vi "Curve Editor(CSM).vi"() -> ()   [LabVIEW 2020, in "Curve Editor.lvlib"]
doc: "------------- lvcsm -------------\n[CSMStates]\nItem 0 = \"Event Structure\"\nItem 1 = \"Idle\"\nItem 2 = \"CSM Documentation\"\nItem 3 = \"VI Reference\"\nItem 4 = \"Error Handler\"\nItem 5 = \"Critical Error\"\nItem 6 = \"Target Timeout Error\"\nItem 7 = \"Target Error\"\nItem 8 = \"Async Response\"\nItem 9 = \"Response\"\nItem 10 = \"Async Message Posted\"\nItem 11 = \"Initialize Core Data\"\nItem 12 = \"Exit\"\nItem 13 = \"Data: Initialize\"\nItem 14 = \"Data: Cleanup\"\nItem 15 = \"Events: Register\"\nItem 16 = \"Events: Unregister\"\nItem 17 = \"UI: Initialize\"\nItem 18 = \"UI: Cursor Set\"\nItem 19 = \"UI: Front Panel State\"\nItem 20 = \"Macro: Initialize\"\nItem 21 = \"Macro: Exit\"\nItem 22 = \"Action: Write File\"\nItem 23 = \"Action: Read File\"\nItem 24 = \"Action: Draw Plot\"\nItem 25 = \"Action: Handle Unsaved Porcess\"\nItem 26 = \"Action: Open File\"\nItem 27 = \"Action: Save File\"\nItem 28 = \"Action: New File\"\nItem 29 = \"Action: Edit Item\"\n\n[CSMStatus]\nItem 0 = \"Error Occurred@Error Handler\""
uses:
  Curve Editor.lvlib
  Curve Editor/User Data--cluster.ctl
  <vilib>/Utility/miscctls.llb/LVPointTypeDef.ctl
  7b0969bd-7955-4222-98c9-53128525ee30.vi
  183b1dfd-394f-40bc-8548-5665fe87f6d3.vi
  54737b30-700e-483c-a5e2-87d6bca6278c.vi
  <userlib>/_NEVSTOP/Communicable State Machine(CSM)/AdvanceAPI/CSM - Revert Arguments-Safe String.vi
  <userlib>/_NEVSTOP/Communicable State Machine(CSM)/_Shared/Trim Single-line Text.vi
  <userlib>/_NEVSTOP/Communicable State Machine(CSM)/AdvanceAPI/CSM - Make String Arguments Safe.vi
  <userlib>/_NEVSTOP/Communicable State Machine(CSM)/AdvanceAPI/CSM - Break Down Multiple States String.vi
  <userlib>/_NEVSTOP/Communicable State Machine(CSM)/AdvanceAPI/CSM - Compact Multiple States.vi
  <userlib>/_NEVSTOP/Communicable State Machine(CSM)/AdvanceAPI/CSM - Keywords.vi
  <userlib>/_NEVSTOP/Communicable State Machine(CSM)/addons/API-String-Arugments-Support/_Support/Data To API String Arguments.vi
  <vilib>/Utility/file.llb/Read Delimited Spreadsheet (string).vi
  <userlib>/_NEVSTOP/Communicable State Machine(CSM)/addons/API-String-Arugments-Support/_Support/Convert API String Arguments to Data(variant).vi
  <userlib>/_NEVSTOP/Communicable State Machine(CSM)/Communicable State Machine.lvlib
panel:
  out "State History":string
  in  "Tab Control":enum32{"Page 1"}(tab)
  in  "动作列表框":i32(listbox) caption="曲线片段"
  in  "循环树形":string(tree) caption="循环编辑"
  in  "打开按钮":bool
  in  "保存按钮":bool
  in  "另存为按钮":bool
  in  "新建按钮":bool
  out "曲线预览":cluster{"X":dbl[], "Y":dbl[]}(graph)
  out "总时长[秒]":dbl format="%.2f"
  in  "Name (\"\" to Use UUID)":string="Curve Editor"
  # "曲线编辑"
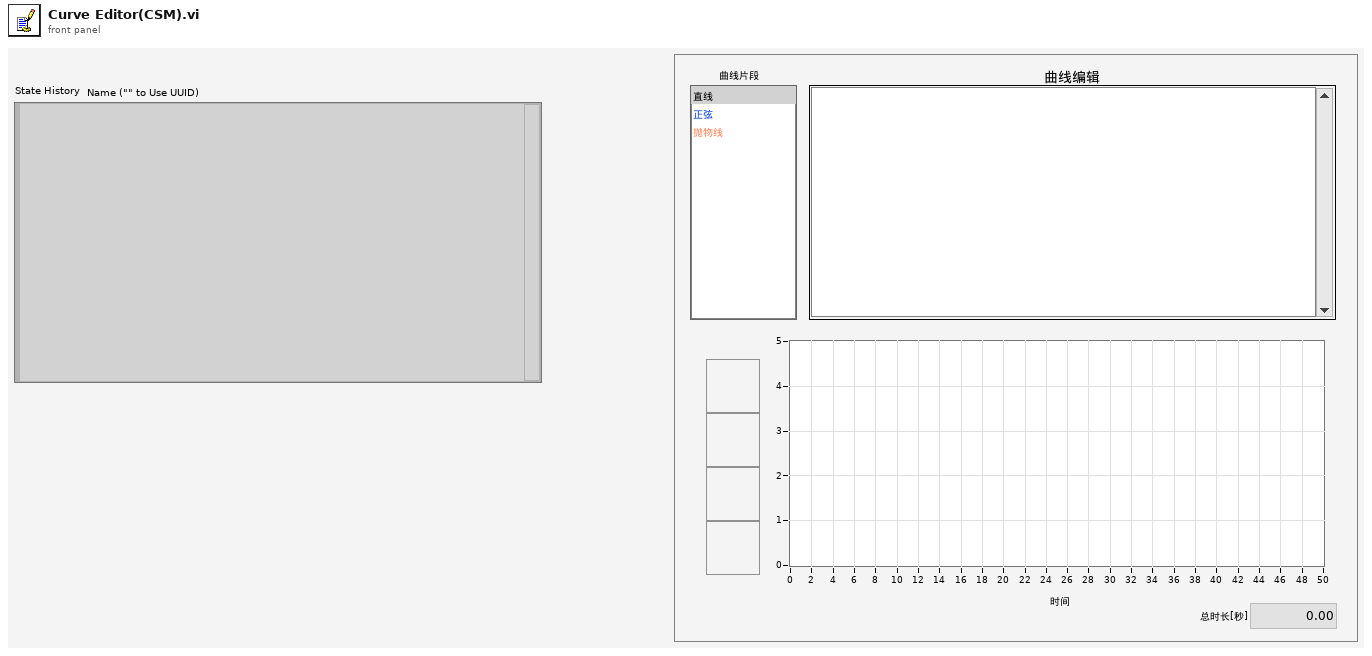
[diagram p1: front panel]
types:
  T1 = enum32{"Invalid", "Standard", "Closed", "Hidden", "Minimized", "Maximized"}
  T2 = enum32{"invalid app kind", "Development System", "Run Time System", "Student Edition", "Embedded LabVIEW", "Evaluation", "Custom"}
  T3 = cluster{"开始路径":path, "默认名称":string, "类型(后缀名)":string, "类型标签":string}
  T4 = typedef "LVPointTypeDef.ctl" = cluster{"Horizontal":i16, "Vertical":i16}
  T5 = enum16{"open", "replace", "create", "open or create", "replace or create", "replace or create with confirmation"}
  T6 = typedef "Communicable State Machine.lvlib/_CSM_Response Source Message.ctl" = cluster{"‘State":string, "’Arguments":string, "’Error":errorcluster}
  T7 = typedef "LVPoint32TypeDef.ctl" = cluster{"Horizontal":i32, "Vertical":i32}
  T8 = typedef "Curve Editor.lvlib/User Data--cluster.ctl" = cluster{"窗体标题":string, "文件参数":cluster{"默认路径":path, "默认名称":string, "类型(后缀名)":string, "类型标签":string}, "颜色符号列表":cluster{"项名":string, "颜色":u32, "符号":i32}[], "循环数组":string[], "文件路径":path, "文件已保存":bool, "存盘提醒":bool}
  T9 = cluster{"Core":cluster{"Current VI Reference":refnum<vi>, "Close Panel on Exit?":bool}, "User Data":T8}
  T10 = cluster{"Current VI Reference":refnum<vi>, "Close Panel on Exit?":bool}
  T11 = cluster{"默认路径":path, "默认名称":string, "类型(后缀名)":string, "类型标签":string}
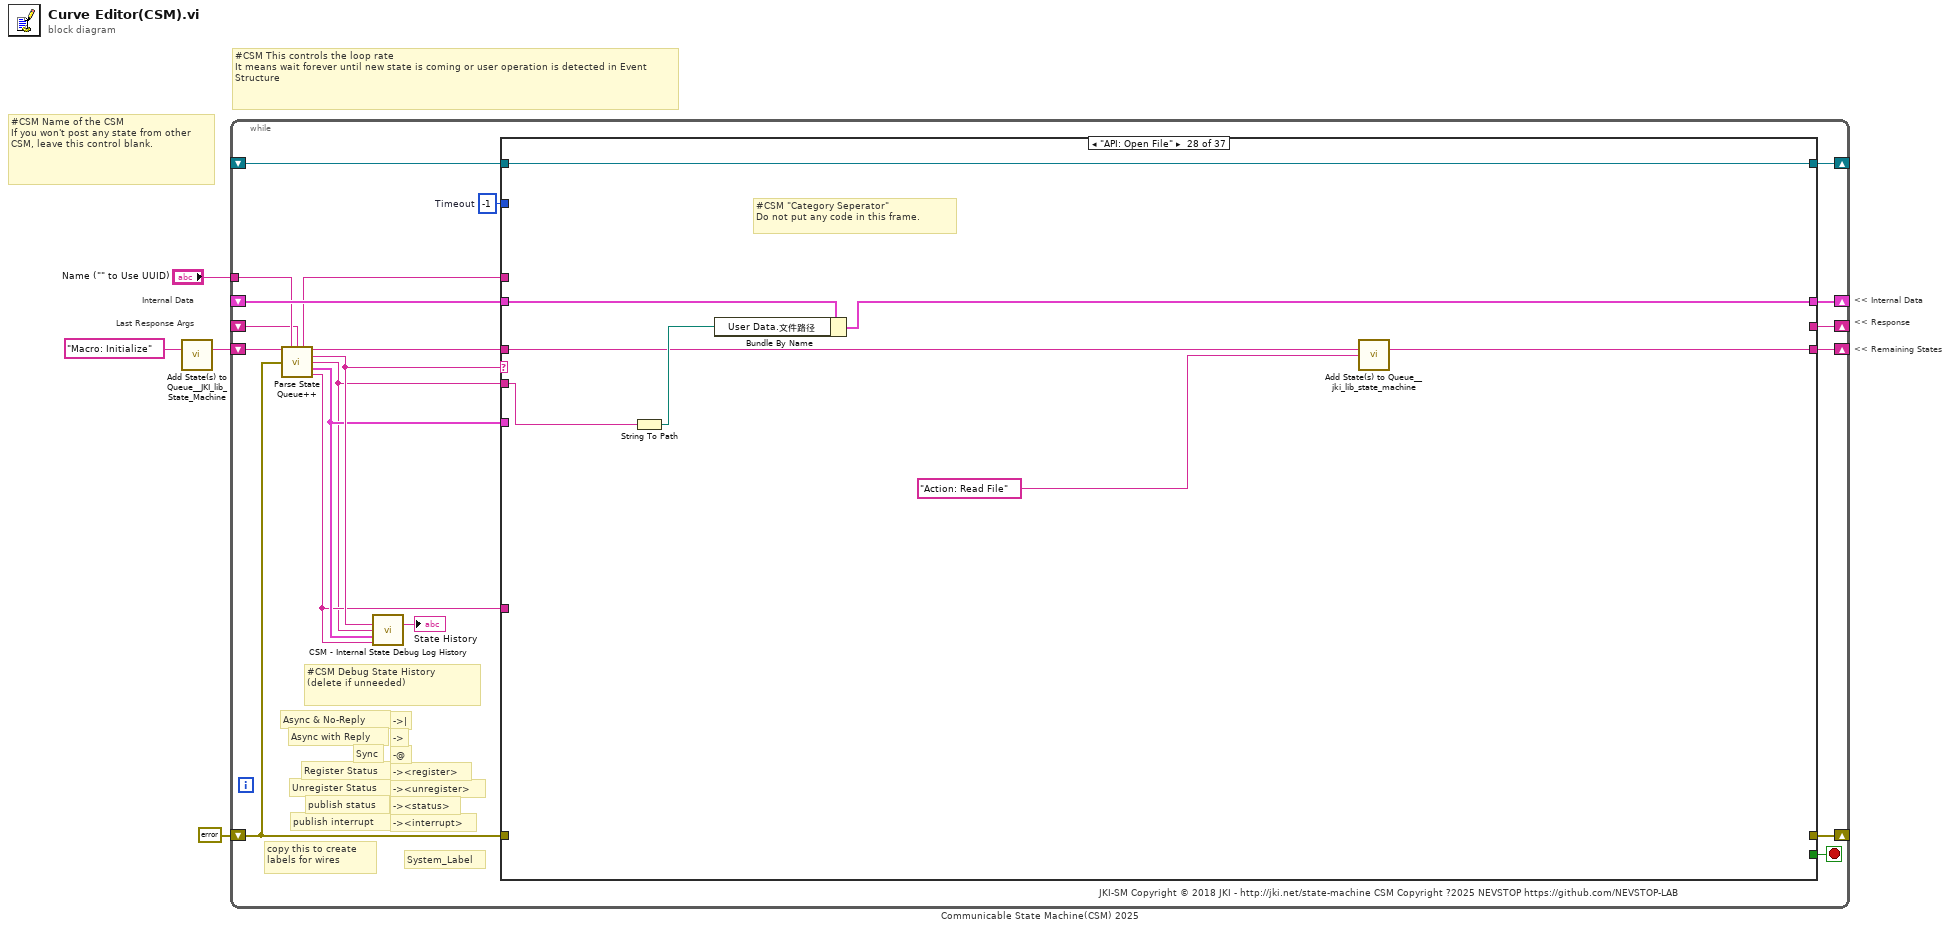
[diagram p0: block diagram]
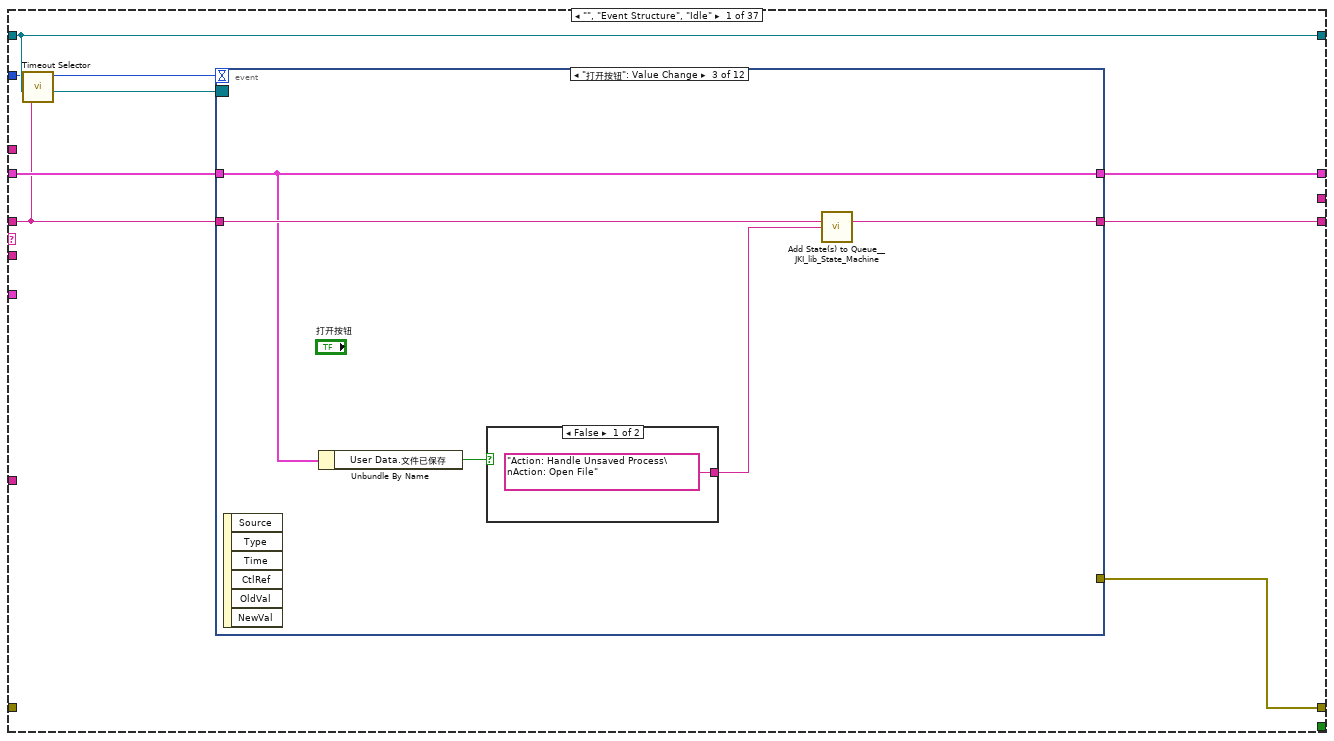
[diagram p2: hidden frame]
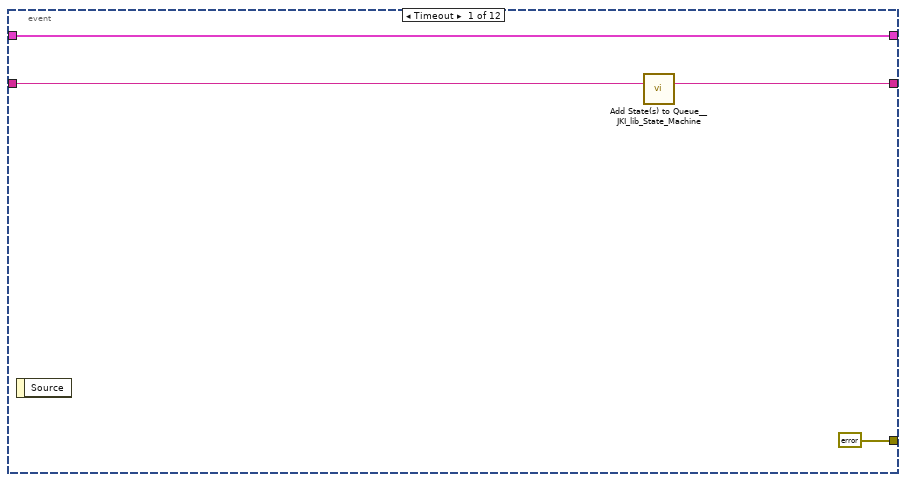
[diagram p3: hidden frame]
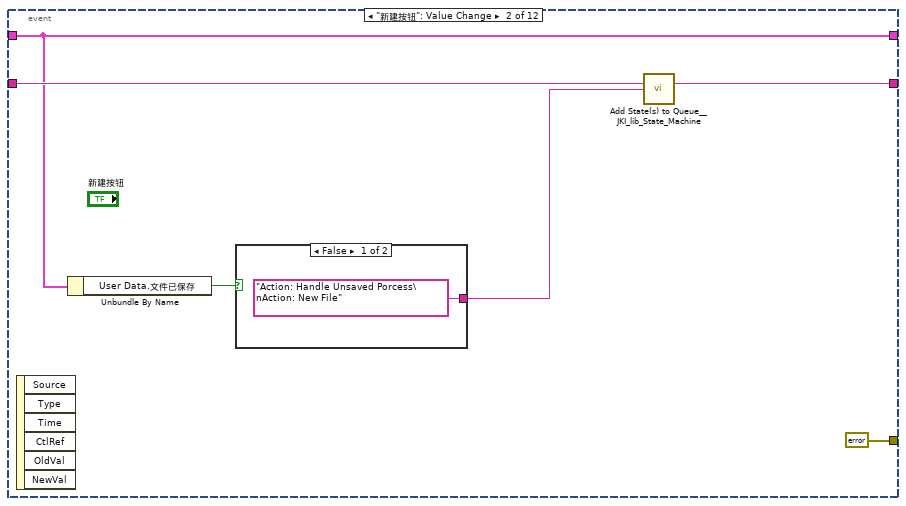
[diagram p4: hidden frame]
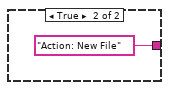
[diagram p5: hidden frame]
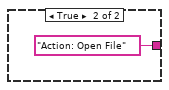
[diagram p6: hidden frame]
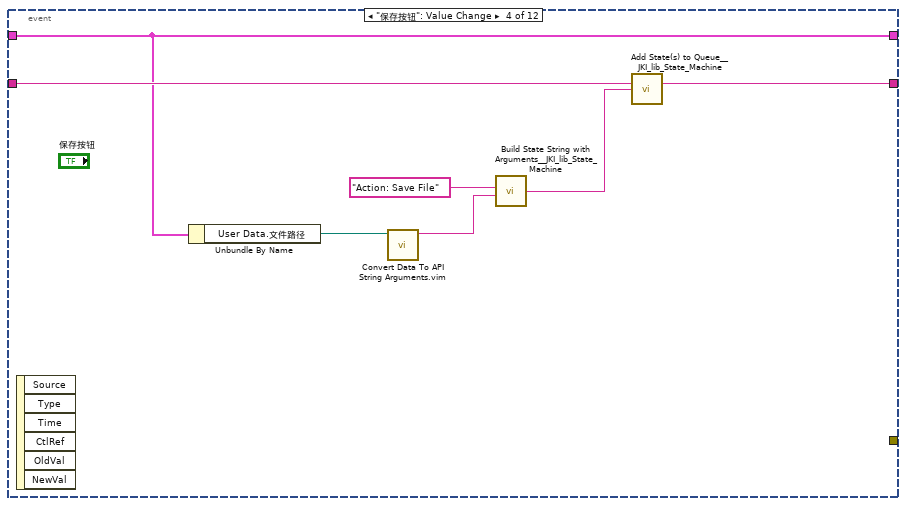
[diagram p7: hidden frame]
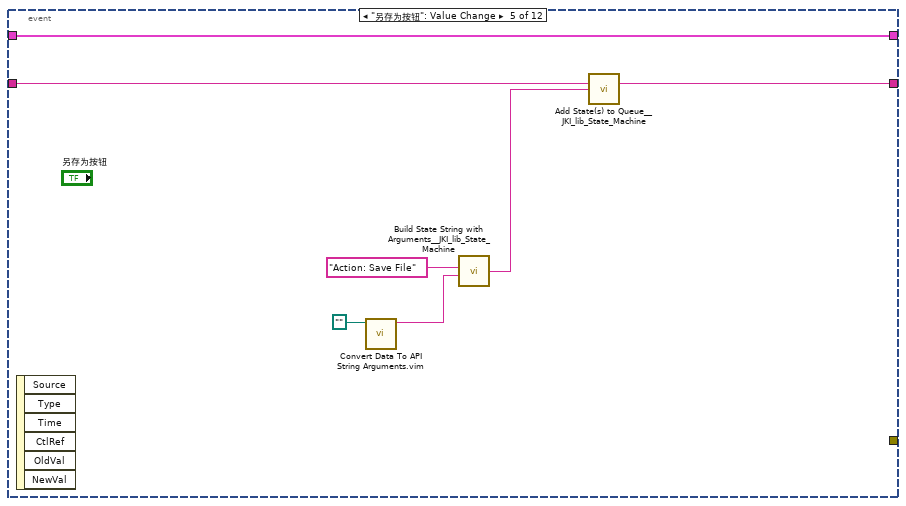
[diagram p8: hidden frame]
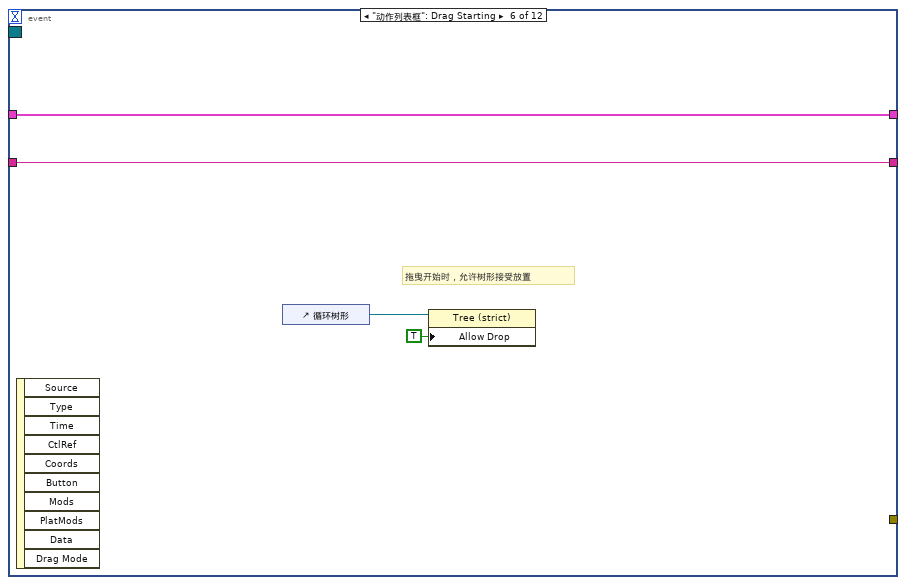
[diagram p9: hidden frame]
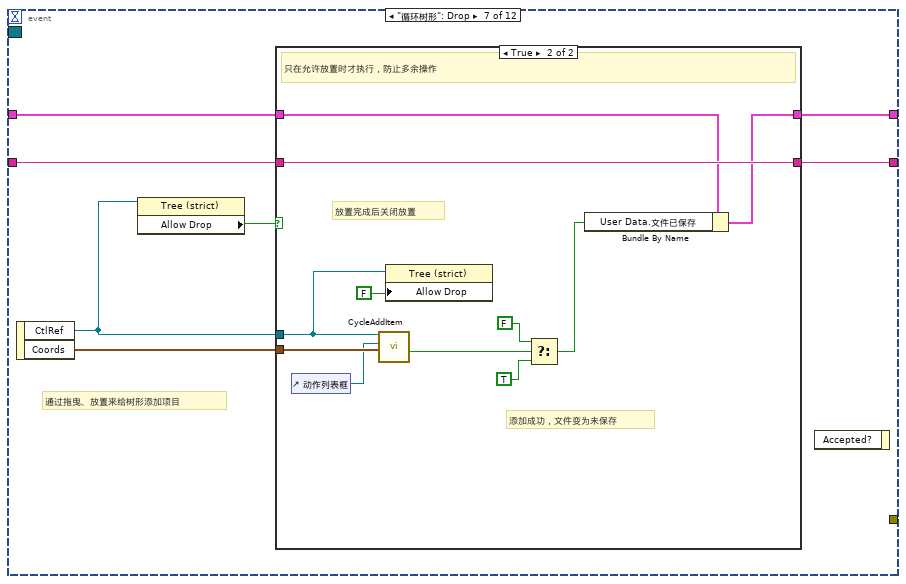
[diagram p10: hidden frame]
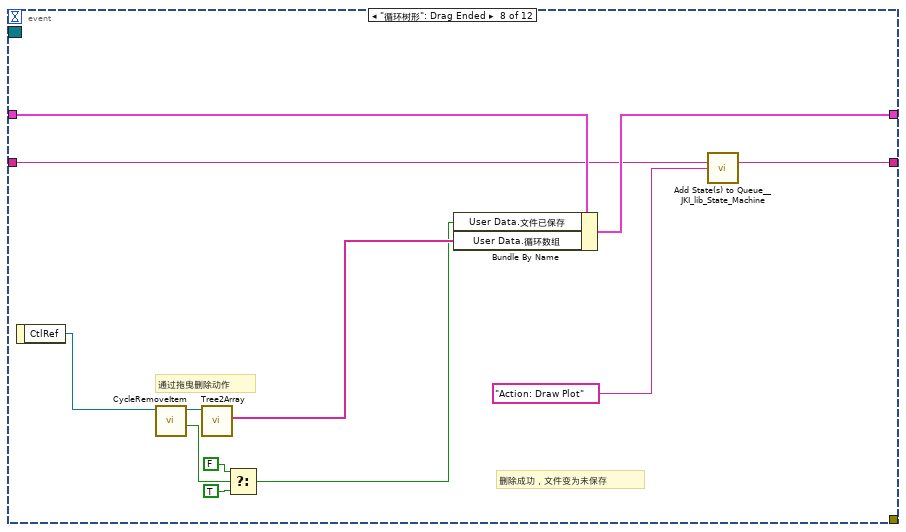
[diagram p12: hidden frame]
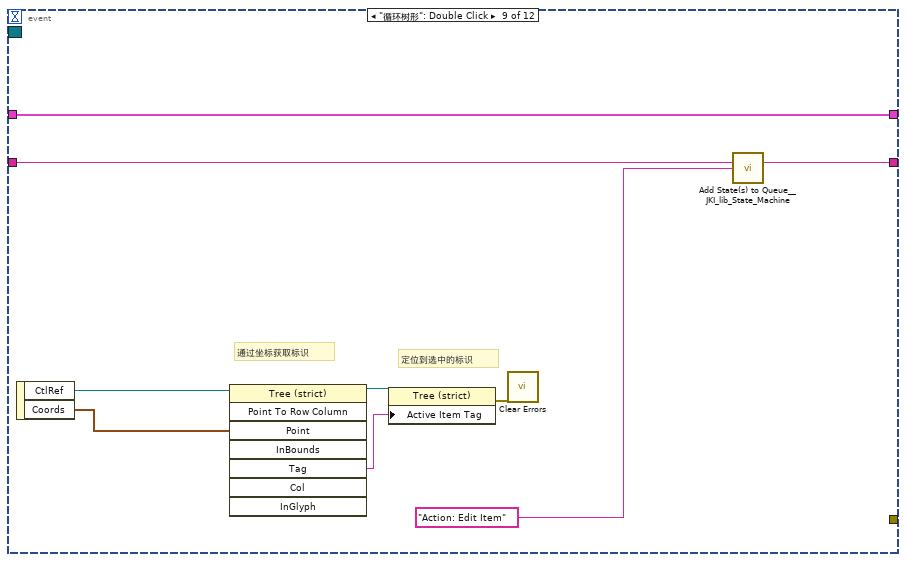
[diagram p13: hidden frame]
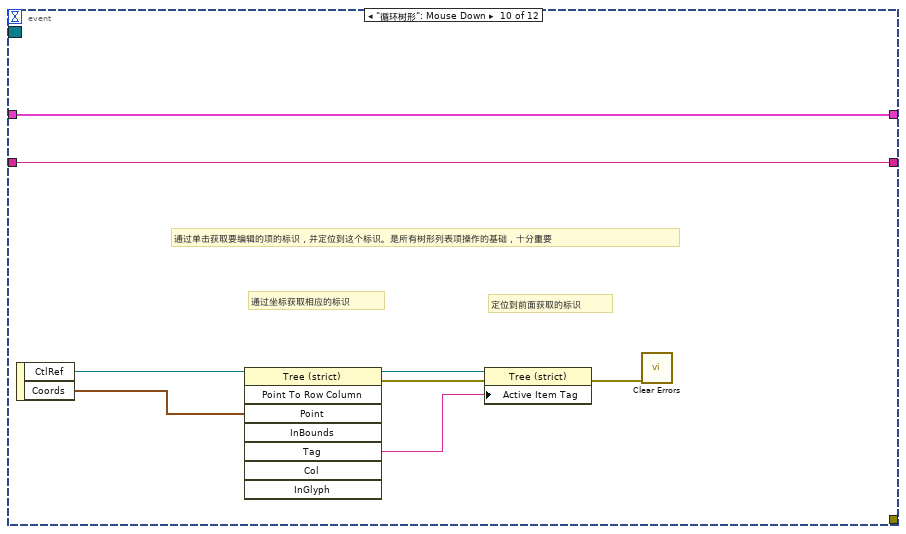
[diagram p14: hidden frame]
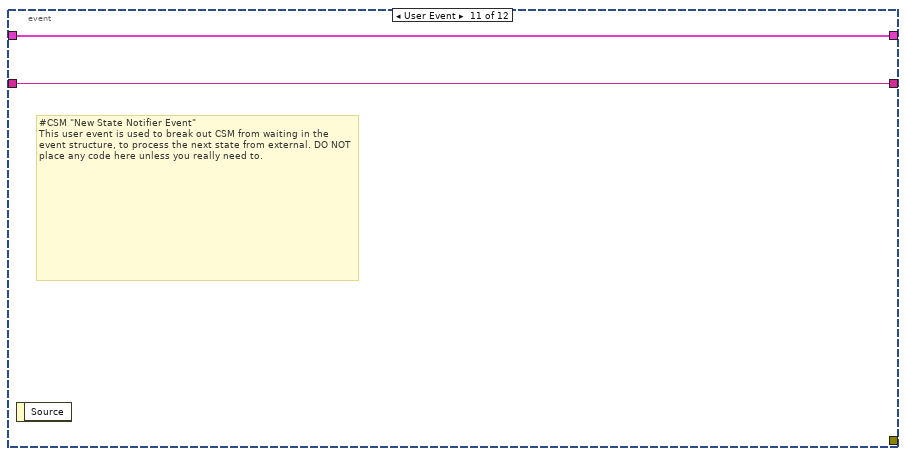
[diagram p15: hidden frame]
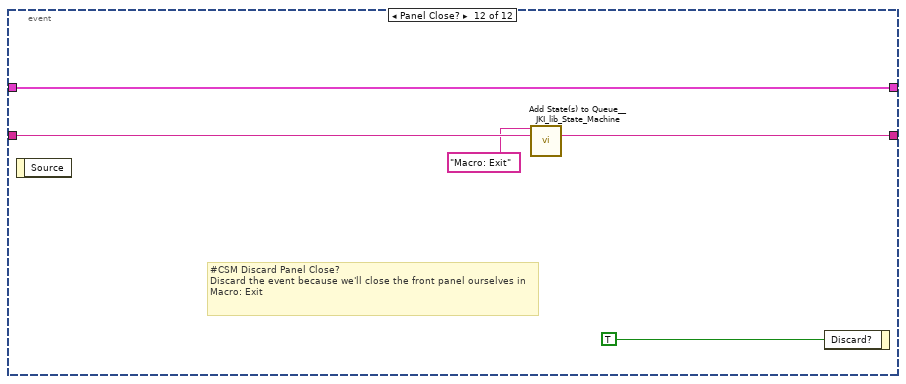
[diagram p16: hidden frame]
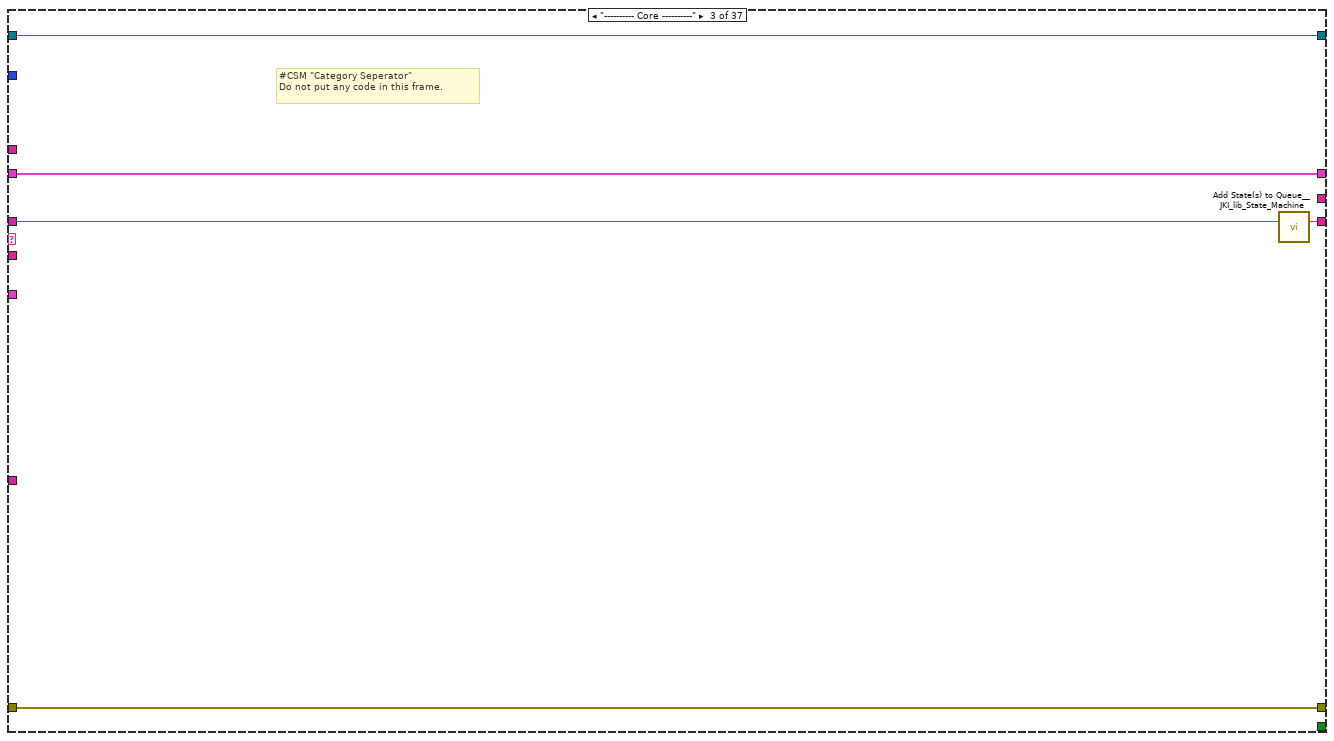
[diagram p18: hidden frame]
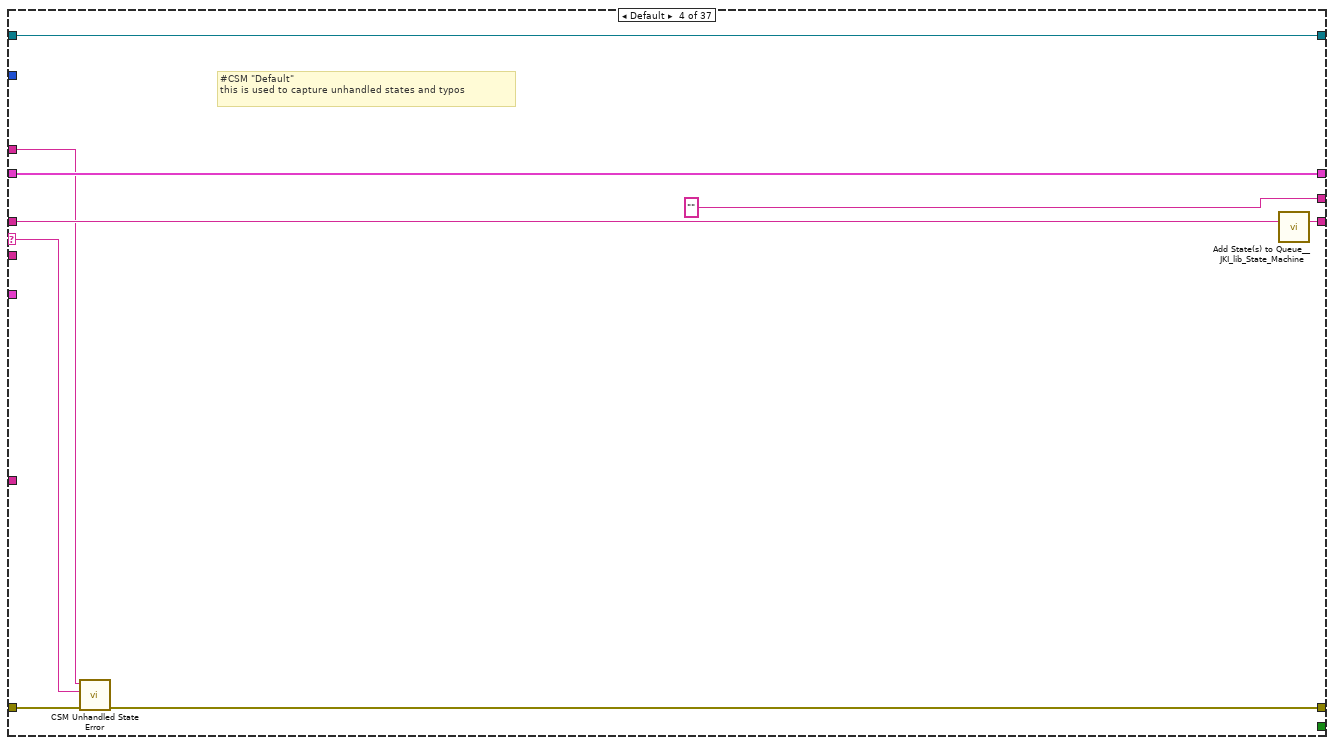
[diagram p19: hidden frame]
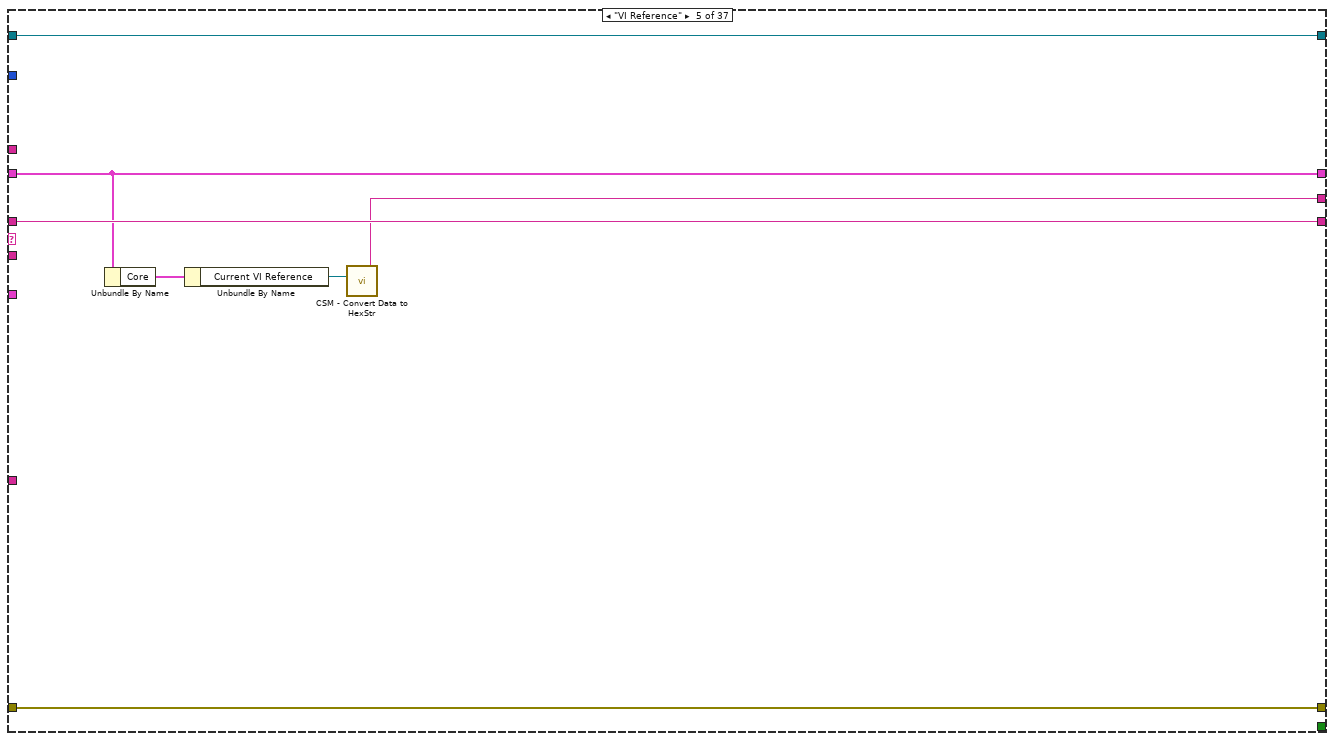
[diagram p20: hidden frame]
diagram:
  # "Last Response Args"
  # "Internal Data"
  # "<< Internal Data"
  # "<< Response"
  # "<< Remaining States"
  # "#CSM Name of the CSM\nIf you won't post any state from other CSM, leave this control blank."
  # "#CSM This controls the loop rate\nIt means wait forever until new state is coming or user operation is detected in Event Structure"
  n1 = call <vilib>:"Add State(s) to Queue__JKI_lib_State_Machine.vi"("State(s) in (\"\")"="Macro: Initialize" ("Init State(\"Macro: Initialize\")")) -> ("States Out"=w1:string)  [unwired: 14 in]
  n2 = while "Communicable State Machine(CSM) 2025" {
    shift-right: [w19] -> _
    shift-left: _ -> [w18]
    shift-right: [w22] -> _
    shift-left: errorcluster {"status"=FALSE, "code"=0, "source"=""} ("error out") -> [w16]
    shift-right: [w21] -> _
    shift-left: w1 -> [w23]
    tunnel: "Name (\"\" to Use UUID)" -> [w12]
    shift-right: [w15] -> _
    shift-left: _ -> [w7]
    shift-right: [w14] -> _
    shift-left: _ -> [w13]
    stop <- w20 stop-if-true
    w17 = -1  # Timeout
    # "#CSM Debug State History\n(delete if unneeded)"
    # "-><interrupt>"
    # "-><status>"
    # "-><unregister>"
    # "-><register>"
    # "-@"
    # "->"
    # "->|"
    # "publish interrupt"
    # "publish status"
    # "Unregister Status"
    # "Register Status"
    # "Sync"
    # "Async with Reply"
    # "Async & No-Reply"
    # "copy this to create labels for wires"
    # "System_Label"
    # "JKI-SM Copyright © 2018 JKI - http://jki.net/state-machine CSM Copyright ?2025 NEVSTOP https://github.com/NEVSTOP-LAB"
    n3 = call <userlib>:"Parse State Queue++.vi"("State Queue"=w23, "Name (\"\" to Use UUID)"=w12, "Response Arguments"=w7, "Previous Error"=w16) -> ("Name Used"=w8:string, "Remaining States"=w24:string, "Current State"=w11:string, "Arguments"=w6:string, "Additional Information"=w10:T6, "Source CSM"=w9:string)  [unwired: 6 in]
    n4 = call <userlib>:"CSM - Internal State Debug Log History.vi"("State"=w11, "Arguments (\"\")"=w6, ">> Response Source Message >>"=w10, "Source (\"\")"=w9) -> ("Debug Log"=→"State History":string)  [unwired: 11 in]
    n5 = case shown="\"API: Open File\"" w11 {
      selector: w11 -> [_ _ _ w136 _ _ _ _ _ _ _ _ _ _ _ _ _ _ _ _ _ _ _ _ _ _ _ _ _ _ _ _ _ _ _ _ _]
      tunnel: w24 -> [w25 w128 w133 w142 w148 w154 w180 w188 w195 w205 w214 w227 w232 w236 w253 w259 w263 w270 w274 w278 w297 w303 w314 w378 w383 w394 w397 w399 w409 w428 w452 w490 w492 w527 w559 w598 w599]
      tunnel: w6 -> [_ _ _ _ _ w152 w176 w183 w191 w199 _ _ _ _ _ _ _ _ _ _ _ w299 w309 _ _ _ _ w403 _ _ _ _ _ _ w556 _ _]
      tunnel: w18 -> [w31 w127 w130 w140 w147 w160 w181 w186 w193 w203 w213 w222 w230 w234 _ w255 w261 w269 w273 w276 w286 w301 w311 w376 w381 w392 w396 w405 w407 w410 w454 w483 w494 w528 w558 w579 w601]
      tunnel: [w30 _ w131 w134 w149 errorcluster {"status"=FALSE, "code"=0, "source"=""} ("error out") w173 w182 w189 w202 _ _ _ _ _ w256 _ w264 w272 _ _ w300 w312 _ _ _ _ _ _ _ _ w491 w501 w537 w566 _ w611] -> w22
      tunnel: w16 -> [_ _ w131 w135 w149 w158 w174 w184 w190 _ _ _ _ _ _ _ _ _ _ _ _ _ _ _ _ _ _ _ _ _ _ w491 w501 w537 w566 _ w611]
      tunnel: [w32 w128 w132 w141 w148 w156 w179 w187 w194 w206 w214 w226 w231 w235 w252 w258 w262 w270 w274 w277 w296 w302 w313 w377 w382 w393 w397 w400 w408 w427 w451 w490 w493 w525 w560 w597 w600] -> w21
      tunnel: [_ _ _ _ _ _ TRUE _ _ _ _ _ TRUE _ _ _ _ _ _ _ _ _ _ _ _ _ _ _ _ _ _ _ _ _ _ _ _] -> w20
      tunnel: [w29 w127 w130 w140 w147 w160 w181 w186 w193 w204 w213 w225 w230 w234 w251 w255 w261 w269 w273 w276 w284 w301 w311 w376 w381 w392 w396 w402 w407 w411 w455 w483 w495 w526 w561 w582 w602] -> w19
      tunnel: w17 -> [w27 _ _ _ _ _ _ _ _ _ _ _ _ _ _ _ _ _ _ _ _ _ _ _ _ _ _ _ _ _ _ _ _ _ _ _ _]
      tunnel: w9 -> [_ _ _ _ _ w151 _ _ _ w200 _ _ _ _ _ _ _ _ _ _ _ _ _ _ _ _ _ _ _ _ _ _ _ _ _ _ _]
      tunnel: w10 -> [_ _ _ _ _ w150 _ _ _ w201 _ _ _ _ _ _ _ _ _ _ _ _ _ _ _ _ _ _ _ _ _ _ _ _ _ _ _]
      tunnel: [_ _ _ "" w143 _ _ _ _ _ _ _ _ _ _ _ _ _ _ _ _ _ _ _ _ _ _ _ _ _ _ _ _ _ _ _ _] -> w15
      tunnel: [w28 w126 w129 w138 w146 w159 w177 w185 w192 w207 w212 w216 w228 w233 w249 w254 w260 w268 w271 w275 w295 w298 w308 w375 w379 w385 w395 w404 w406 w426 w464 w489 w500 w536 w565 w596 w610] -> w14
      tunnel: w13 -> [w28 w126 w129 w138 w146 w159 w177 w185 w192 w207 w212 w216 w228 w233 w249 w254 w260 _ w271 w275 w295 w298 w308 w375 w379 w385 w395 w404 w406 w426 w464 w489 w500 w536 w565 w596 w610]
      tunnel: w8 -> [_ _ _ w137 _ _ w175 _ _ _ _ _ _ _ _ _ _ w267 _ _ _ _ _ _ _ _ _ _ _ _ _ _ _ _ _ _ _]
      frame "", "Event Structure", "Idle" {
        n6 = call <userlib>:"Timeout Selector.vi"("Remaining States"=w25, "Timeout Expected"=w27) -> ("Timeout"=w26:i32)  [unwired: 5 in]
        n7 = event shown="[2] \"打开按钮\": Value Change" {
          selector: w28 -> [_ _ _ _ _ _ _ _ _ _ _ _]
          dyn-events: _ -> [_ _ _ _ _ _ _ _ _ _ _ _]
          timeout: w26 -> [_ _ _ _ _ _ _ _ _ _ _ _]
          tunnel: w25 -> [w36 w42 w49 w57 w63 w69 w70 w91 w103 w118 w119 w125]
          tunnel: [w35 w41 w48 w58 w64 w69 w71 w92 w104 w118 w119 w124] -> w32
          tunnel: w31 -> [w34 w38 w47 w55 w65 w68 w73 w101 w110 w117 w120 w123]
          tunnel: [errorcluster {"status"=FALSE, "code"=0, "source"=""} ("error out") errorcluster {"status"=FALSE, "code"=0, "source"=""} ("error out") _ _ _ _ _ _ _ _ _ _] -> w30
          tunnel: [w34 w38 w47 w55 w65 w68 w72 w100 w110 w117 w120 w123] -> w29
          event Timeout {
            n8 = event-data() -> ()  [unwired: 1 in, 1 out]
            n9 = call <vilib>:"Add State(s) to Queue__JKI_lib_State_Machine.vi"("State(s) in (\"\")"=w36) -> ("States Out"=w35:string)  [unwired: 14 in]
          }
          event "新建按钮": Value Change {
            n10 = event-data() -> ()  [unwired: 1 in, 6 out]
            n11 = Unbundle By Name(w38) -> ("User Data.文件已保存"=w39:bool)
            n12 = case shown="False" w39 {
              tunnel: ["Action: Handle Unsaved Porcess\nAction: New File" "Action: New File"] -> w37
              frame False {
              }
              frame True {
              }
            }
            n13 = call <vilib>:"Add State(s) to Queue__JKI_lib_State_Machine.vi"("State(s) in (\"\")"=w42, "State(s) at Back (\"\")"=w37) -> ("States Out"=w41:string)  [unwired: 13 in]
          }
          event "打开按钮": Value Change {
            n14 = event-data() -> ()  [unwired: 1 in, 6 out]
            n15 = Unbundle By Name(w47) -> ("User Data.文件已保存"=w46:bool)
            n16 = case shown="False" w46 {
              tunnel: ["Action: Handle Unsaved Process\nAction: Open File" "Action: Open File"] -> w45
              frame False {
              }
              frame True {
              }
            }
            n17 = call <vilib>:"Add State(s) to Queue__JKI_lib_State_Machine.vi"("State(s) in (\"\")"=w49, "State(s) at Back (\"\")"=w45) -> ("States Out"=w48:string)  [unwired: 13 in]
          }
          event "保存按钮": Value Change {
            n18 = event-data() -> ()  [unwired: 1 in, 6 out]
            n19 = Unbundle By Name(w55) -> ("User Data.文件路径"=w54:path)
            n20 = call "Convert Data To API String Arguments.vim"("Data"=w54) -> ("API String"=w53:string)  [unwired: 7 in, 1 out]
            n21 = call <vilib>:"Build State String with Arguments__JKI_lib_State_Machine.vi"("Arguments (\"\")"=w53, "State"="Action: Save File" ("State(s) at Back (\"\")")) -> ("State with Arguments"=w52:string)  [unwired: 4 in]
            n22 = call <vilib>:"Add State(s) to Queue__JKI_lib_State_Machine.vi"("State(s) in (\"\")"=w57, "State(s) at Back (\"\")"=w52) -> ("States Out"=w58:string)  [unwired: 13 in]
          }
          event "另存为按钮": Value Change {
            n23 = event-data() -> ()  [unwired: 1 in, 6 out]
            n24 = call "Convert Data To API String Arguments.vim"("Data"=path "") -> ("API String"=w59:string)  [unwired: 7 in, 1 out]
            n25 = call <vilib>:"Build State String with Arguments__JKI_lib_State_Machine.vi"("Arguments (\"\")"=w59, "State"="Action: Save File" ("State(s) at Back (\"\")")) -> ("State with Arguments"=w61:string)  [unwired: 4 in]
            n26 = call <vilib>:"Add State(s) to Queue__JKI_lib_State_Machine.vi"("State(s) in (\"\")"=w63, "State(s) at Back (\"\")"=w61) -> ("States Out"=w64:string)  [unwired: 13 in]
          }
          event "动作列表框": Drag Starting {
            # "拖曳开始时，允许树形接受放置"
            n27 = event-data() -> ()  [unwired: 1 in, 10 out]
            n28 = control-ref of="循环树形"() -> (w66:refnum<vi>)
            n29 = property class="Tree (strict)"(reference=w66, "Allow Drop"=TRUE ("拖曳/放置:允许放置")) -> ()  [unwired: 1 in, 2 out]
          }
          event "循环树形": Drop {
            # "通过拖曳、放置来给树形添加项目"
            n30 = event-data() -> ("CtlRef"=w75:refnum<vi>, "Coords"=w74:T7)  [unwired: 1 in]
            n31 = property class="Tree (strict)"(reference=w75) -> ("Allow Drop"=w76:bool)  [unwired: 1 in, 2 out]
            n32 = case shown="True" w76 {
              tunnel: w74 -> [_ w89]
              tunnel: w75 -> [_ w86]
              tunnel: w73 -> [w78 w81]
              tunnel: [w78 w79] -> w72
              tunnel: [w77 w82] -> w71
              tunnel: w70 -> [w77 w82]
              frame False {
              }
              frame True {
                # "添加成功，文件变为未保存"
                # "放置完成后关闭放置"
                # "只在允许放置时才执行，防止多余操作"
                n33 = control-ref of="动作列表框"() -> (w88:refnum<vi>)
                n34 = call "CycleAddItem.vi"("Coords"=w89, "动作列表框"=w88, "TreeControl输入"=w86) -> ("添加成功"=w83:bool)  [unwired: 6 in, 2 out]
                n35 = property class="Tree (strict)"(reference=w86, "Allow Drop"=FALSE ("拖曳/放置:允许放置")) -> ()  [unwired: 1 in, 2 out]
                n36 = Select(t=FALSE, s=w83, f=TRUE) -> (s? t:f=w80:bool)
                n37 = Bundle By Name(cluster=w81, "User Data.文件已保存"=w80) -> (w79:T9)
              }
            }
            n38 = event-data() -> ()  [unwired: 2 in, 1 out]
          }
          event "循环树形": Drag Ended {
            # "删除成功，文件变为未保存"
            # "通过拖曳删除动作"
            n39 = event-data() -> ("CtlRef"=w95:refnum<vi>)  [unwired: 1 in]
            n40 = call "CycleRemoveItem.vi"("TreeControl输入"=w95) -> ("删除成功"=w98:bool, "TreeControl输出"=w99:refnum<vi>)  [unwired: 8 in, 1 out]
            n41 = call "Tree2Array.vi"("TreeControl输入"=w99) -> ("循环数组"=w94:string[])  [unwired: 9 in, 1 out]
            n42 = Select(t=FALSE, s=w98, f=TRUE) -> (s? t:f=w93:bool)
            n43 = Bundle By Name(cluster=w101, "User Data.文件已保存"=w93, "User Data.循环数组"=w94) -> (w100:T9)
            n44 = call <vilib>:"Add State(s) to Queue__JKI_lib_State_Machine.vi"("State(s) in (\"\")"=w91, "State(s) at Back (\"\")"="Action: Draw Plot" ("State(s) at Back (\"\")")) -> ("States Out"=w92:string)  [unwired: 13 in]
          }
          event "循环树形": Double Click {
            # "定位到选中的标识"
            # "通过坐标获取标识"
            n45 = event-data() -> ("CtlRef"=w105:refnum<vi>, "Coords"=w106:T7)  [unwired: 1 in]
            n46 = invoke class="Tree (strict)" method="Point To Row Column"(reference=w105, "Point"=w106) -> (reference out=w107:refnum<vi>, "Tag"=w108:string)  [unwired: 6 in, 6 out]
            n47 = property class="Tree (strict)"(reference=w107, "Active Item Tag"=w108) -> (error out=w109:errorcluster)  [unwired: 1 in, 1 out]
            n48 = call <vilib>:"Clear Errors.vi"("error in (no error)"=w109) -> ()  [unwired: 5 in, 2 out]
            n49 = call <vilib>:"Add State(s) to Queue__JKI_lib_State_Machine.vi"("State(s) in (\"\")"=w103, "State(s) at Back (\"\")"="Action: Edit Item" ("State(s) at Back (\"\")")) -> ("States Out"=w104:string)  [unwired: 13 in]
          }
          event "循环树形": Mouse Down {
            # "定位到前面获取的标识"
            # "通过坐标获取相应的标识"
            # "通过单击获取要编辑的项的标识，并定位到这个标识。是所有树形列表项操作的基础，十分重要"
            n50 = event-data() -> ("CtlRef"=w112:refnum<vi>, "Coords"=w111:T7)  [unwired: 1 in]
            n51 = invoke class="Tree (strict)" method="Point To Row Column"(reference=w112, "Point"=w111) -> (reference out=w113:refnum<vi>, error out=w115:errorcluster, "Tag"=w114:string)  [unwired: 6 in, 5 out]
            n52 = property class="Tree (strict)"(reference=w113, error in=w115, "Active Item Tag"=w114) -> (error out=w116:errorcluster)  [unwired: 1 out]
            n53 = call <vilib>:"Clear Errors.vi"("error in (no error)"=w116) -> ()  [unwired: 5 in, 2 out]
          }
          event User Event {
            # "#CSM \"New State Notifier Event\"\nThis user event is used to break out CSM from waiting in the event structure, to process the next state from external. DO NOT place any code here unless you really need to."
            n54 = event-data() -> ()  [unwired: 1 in, 1 out]
          }
          event Panel Close? {
            # "#CSM Discard Panel Close?\nDiscard the event because we'll close the front panel ourselves in Macro: Exit"
            n55 = event-data() -> ()  [unwired: 1 in, 1 out]
            n56 = call <vilib>:"Add State(s) to Queue__JKI_lib_State_Machine.vi"("State(s) in Front (\"\")"="Macro: Exit", "State(s) in (\"\")"=w125) -> ("States Out"=w124:string)  [unwired: 13 in]
            n57 = event-data("Discard?"=TRUE) -> ()  [unwired: 1 in, 1 out]
          }
        }
      }
      frame "CSM Documentation" {
        # "#CSM \"Documentation\"\nCase for holding CSM Documenation"
      }
      frame "---------- Core ----------" {
        # "#CSM \"Category Seperator\"\nDo not put any code in this frame."
        n58 = call <vilib>:"Add State(s) to Queue__JKI_lib_State_Machine.vi"("State(s) in (\"\")"=w133) -> ("States Out"=w132:string)  [unwired: 14 in]
      }
      frame Default {
        # "#CSM \"Default\"\nthis is used to capture unhandled states and typos"
        n59 = call <userlib>:"CSM Unhandled State Error.vi"("error in (no error)"=w135, "Undefined State"=w136, "CSM Name"=w137) -> ("error out"=w134:errorcluster)  [unwired: 8 in]
        n60 = call <vilib>:"Add State(s) to Queue__JKI_lib_State_Machine.vi"("State(s) in (\"\")"=w142) -> ("States Out"=w141:string)  [unwired: 14 in]
      }
      frame "VI Reference" {
        n61 = Unbundle By Name(w147) -> ("Core"=w145:T10)
        n62 = Unbundle By Name(w145) -> ("Current VI Reference"=w144:refnum<vi>)
        n63 = call <userlib>:"CSM - Convert Data to HexStr.vi"("Variant"=w144) -> ("HEX String (0-9,A-F)"=w143:string)  [unwired: 8 in]
      }
      frame "Error Handler" {
        # "#CSM Disable this error dialog if you need"
        # "#CSM \"Error Handler\"\nYou can also output any states to clean-up after errors occur"
        # "Clear error"
        n64 = case shown="Error" w158 {
          selector: w158 -> [_ w167]
          tunnel: [w165 w169] -> w155
          tunnel: w154 -> [w165 w168]
          tunnel: [w164 w167] -> w153
          tunnel: w152 -> [w166 _]
          tunnel: w151 -> [_ _]
          tunnel: w150 -> [_ _]
          frame No Error {
            n65 = call <userlib>:"CSM - Convert Argument to Error.vi"("Argument"=w166) -> ("Error"=w164:errorcluster)  [unwired: 4 in]
            n66 = flat-sequence {
              frame #0 {
                # "#CSM External Error Handler Case\nUsually, it's because This CSM register others' \"Error Occurred\" status with \"Error Handler\". If other CSM have any error, the error will be passed here for central handling."
              }
            }
          }
          frame Error {
            # "#CSM Internal Error Handler Case \nIf any error Occurred, \"Error Occurred\" \nstatus update will be broadcasted to system.\nParameter is Error Cluster."
            n67 = call <userlib>:"CSM - Convert Error to Argument.vi"("Error"=w167) -> ("Argument"=w171:string)  [unwired: 4 in]
            n68 = call <vilib>:"Build State String with Arguments__JKI_lib_State_Machine.vi"("Arguments (\"\")"=w171, "State"="Error Occurred" ("Status with Arguments")) -> ("State with Arguments"=w170:string)  [unwired: 4 in]
            n69 = call <userlib>:"CSM - Broadcast Status Change.vi"("Status With Arguments"=w170, "State Queue"=w168) -> ("Remaining States"=w169:string)  [unwired: 13 in]
          }
        }
        n70 = disable-structure shown="Enabled" {
          disable-tunnel: w153 -> [w162 w163]
          frame Enabled {
            # "Unhandled Error -- Display it"
            n71 = call <vilib>:"General Error Handler.vi"("error in (no error)"=w162) -> ()  [unwired: 10 in, 5 out]
          }
          frame Disabled {
            n72 = call <vilib>:"Clear Errors.vi"("error in (no error)"=w163) -> ()  [unwired: 5 in, 2 out]
          }
        }
        n73 = call <vilib>:"Add State(s) to Queue__JKI_lib_State_Machine.vi"("State(s) in Front (\"\")"="// Post Error States", "State(s) in (\"\")"=w155) -> ("States Out"=w156:string)  [unwired: 13 in]
      }
      frame "Critical Error" {
        # "#CSM \"Critical Error\"\nWhen any un-recoverable error occurs, CSM goes into this case."
        # "#CSM Stop in Critical Error\nWhen Critical Error occurs, Stop the loop immediately. Do NOT change this unless you fully understand the impact."
        n74 = call <userlib>:"CSM Critical Error.vi"("error in (no error)"=w174, "Arugments (As Reason)"=w176, "CSM Name"=w175) -> ("error out"=w173:errorcluster)  [unwired: 8 in]
        n75 = call <vilib>:"Add State(s) to Queue__JKI_lib_State_Machine.vi"("State(s) in (\"\")"=w180) -> ("States Out"=w179:string)  [unwired: 14 in]
      }
      frame "Target Timeout Error" {
        # "#CSM \"Target Timeout Error\"\nWhen This CSM could not get the sync-call response in time, This CSM goes into this case."
        n76 = call <userlib>:"CSM Target Timeout Error.vi"("error in (no error)"=w184, "Arguments (As CSM Name)"=w183) -> ("error out"=w182:errorcluster)  [unwired: 9 in]
        n77 = call <vilib>:"Add State(s) to Queue__JKI_lib_State_Machine.vi"("State(s) in (\"\")"=w188) -> ("States Out"=w187:string)  [unwired: 14 in]
      }
      frame "Target Error" {
        # "#CSM \"Target Error\"\nWhen This CSM try to communicate with an un-existed CSM, This CSM goes into this case."
        n78 = call <userlib>:"CSM Target Error.vi"("error in (no error)"=w190, "Arguments (As CSM Name)"=w191) -> ("error out"=w189:errorcluster)  [unwired: 9 in]
        n79 = call <vilib>:"Add State(s) to Queue__JKI_lib_State_Machine.vi"("State(s) in (\"\")"=w195) -> ("States Out"=w194:string)  [unwired: 14 in]
      }
      frame "Async Response", "Response" {
        # "#CSM \"Async Response\"\nHandle Async-call Response (\"Async Response\" for ->)"
        # "#CSM \"Response\"\nHandle Sync-call Response (\"Response\" for -@)"
        n80 = Unbundle(w201) -> ("‘State"=w198:string, "’Arguments"=w197:string, "’Error"=w196:errorcluster)
        n81 = case shown="Default" w198 {
          tunnel: [w208] -> w206
          tunnel: w205 -> [w209]
          tunnel: [w211] -> w204
          tunnel: w203 -> [w211]
          tunnel: [w210] -> w202
          tunnel: w196 -> [w210]
          tunnel: w200 -> [_]
          tunnel: w199 -> [_]
          tunnel: w197 -> [_]
          frame Default {
            # "#CSM Response Comments\nAfter Message is executed, CSM goes to this state for receive the response.\n    For Async Message(->), \"Async Response\" is used. This CSM will goes to \"Async Message Posted\" immediately and receive the \"Async Response\" after the callee finishes the message.\n    For Sync Message(@),  This CSM will wait until the message is done and immediately goes to \"Response\""
            n82 = call <vilib>:"Add State(s) to Queue__JKI_lib_State_Machine.vi"("State(s) in (\"\")"=w209) -> ("States Out"=w208:string)  [unwired: 14 in]
          }
        }
      }
      frame "Async Message Posted" {
        # "#CSM \"Async Message Posted\"\nAfter Async Message is posted (-> or ->| ), CSM goes to this state for post-action.\nYou can use Argument - State to tell which Async Message is called."
      }
      frame "Initialize Core Data" {
        # "#CSM \"Initialize Core Data\"\nThis is used to determine panel behavior on exit"
        # "originally closed?"
        # "exe?"
        # "If panel starts closed or is an EXE, then close it when we exit"
        n83 = property class="VI"() -> ("FP.State"=w219:T1)  [unwired: 2 in, 2 out]
        n84 = control-ref of="Current VI Reference"() -> (w220:refnum<vi>)
        n85 = property class="App"() -> ("App.Kind"=w224:T2)  [unwired: 2 in, 2 out]
        n86 = Equal?(x=w219, y=T1."Closed" ("Front Panel Window:State")) -> (x = y?=w217:bool)
        n87 = Equal?(x=w224, y=T2."Run Time System" ("Application:Kind")) -> ()  [unwired: 1 out]
        n88 = Or(x=w217, y=TRUE) -> (x .or. y?=w221:bool)
        n89 = Bundle By Name(cluster=w222, "Core.Current VI Reference"=w220, "Core.Close Panel on Exit?"=w221) -> (w225:T9)
        n90 = call <vilib>:"Add State(s) to Queue__JKI_lib_State_Machine.vi"("State(s) in (\"\")"=w227) -> ("States Out"=w226:string)  [unwired: 14 in]
      }
      frame "Exit" {
        # "#CSM \"Exit\"\nCase for exiting the loop. No errors that occur here will be handled."
        n91 = call <vilib>:"Add State(s) to Queue__JKI_lib_State_Machine.vi"("State(s) in (\"\")"=w232) -> ("States Out"=w231:string)  [unwired: 14 in]
      }
      frame "---------- Data ----------" {
        # "#CSM \"Category Seperator\"\nDo not put any code in this frame."
        n92 = call <vilib>:"Add State(s) to Queue__JKI_lib_State_Machine.vi"("State(s) in (\"\")"=w236) -> ("States Out"=w235:string)  [unwired: 14 in]
      }
      frame "Data: Initialize" {
        w248 = T8 {"窗体标题"="", "文件参数"={"默认路径"=path "", "默认名称"="", "类型(后缀名)"="", "类型标签"=""}, "颜色符号列表"=[], "循环数组"=[], "文件路径"=path "", "文件已保存"=FALSE, "存盘提醒"=FALSE}  # User Data
        w250 = T10 {"Current VI Reference"=refnum, "Close Panel on Exit?"=FALSE}  # Core
        # "#CSM  do not delete - used by framework"
        # "#CSM Expand Bundle to add new data elements to shift register data."
        # "#CSM Data names and types of shift register data are defined by this bundle."
        # "#CSM \"Data: Initialize\"\nInitialize the shift-register data, here.\n(data names are defined by what you wire into the bundle function)"
        n93 = call <vilib>:"Application Directory.vi"() -> ("Application Directory"=w237:path)
        n94 = Bundle By Name(cluster=T3 {"开始路径"=path "", "默认名称"="", "类型(后缀名)"="", "类型标签"=""} ("文件参数"), "开始路径"=w237, "默认名称"="新曲线" ("文件_默认文件名"), "类型(后缀名)"="*.cuv" ("文件_后缀名"), "类型标签"="曲线配置文件" ("文件_类型标签")) -> (w242:T3)
        n95 = Bundle By Name(cluster=w248, "文件参数"=w242, "循环数组"=string[] [], "文件路径"=path "", "文件已保存"=TRUE, "存盘提醒"=TRUE) -> (w247:T8)
        n96 = Bundle("Core"=w250, "User Data"=w247) -> (w251:T9)  [unwired: 1 in]
        n97 = call <vilib>:"Add State(s) to Queue__JKI_lib_State_Machine.vi"("State(s) in (\"\")"=w253) -> ("States Out"=w252:string)  [unwired: 14 in]
      }
      frame "Data: Cleanup" {
        # "#CSM \"Data: Cleanup\"\nCleanup any data and references, here.\n(this is called automatically, by the Macro: Exit)"
        n98 = Unbundle By Name(w255) -> ("Core.Current VI Reference"=w257:refnum<vi>)
        n99 = Close Reference(reference=w257) -> (error out=w256:errorcluster)  [unwired: 1 in]
        n100 = call <vilib>:"Add State(s) to Queue__JKI_lib_State_Machine.vi"("State(s) in (\"\")"=w259) -> ("States Out"=w258:string)  [unwired: 14 in]
      }
      frame "---------- Events ----------" {
        # "#CSM \"Category Seperator\"\nDo not put any code in this frame."
        n101 = call <vilib>:"Add State(s) to Queue__JKI_lib_State_Machine.vi"("State(s) in (\"\")"=w263) -> ("States Out"=w262:string)  [unwired: 14 in]
      }
      frame "Events: Register" {
        # "#CSM \"Events: Register\"\nRegister user event. New Message Event is registered to break CSM waiting in event structure by default."
        # "#CSM Register New Message Event\nRegister message event to break Waiting in Event structure."
        n102 = call <userlib>:"CSM - Get New State Notifier Event.vi"("Name (\"\" to Use UUID)"=w267) -> ("error out"=w265:errorcluster, "New State Notifier Event"=w266:refnum<user-event>)  [unwired: 9 in]
        n103 = register-events(error in=w265, w266) -> (reference out=w268:refnum<event-registration>, error out=w264:errorcluster)  [unwired: 1 in]
      }
      frame "Events: Unregister" {
        # "#CSM \"Events: Unregister\"\nUnregister user event."
        n104 = Unregister For Events(event registration refnum=w271) -> (error out=w272:errorcluster)  [unwired: 1 in]
      }
      frame "---------- UI ----------" {
        # "#CSM \"Category Seperator\"\nDo not put any code in this frame."
        n105 = call <vilib>:"Add State(s) to Queue__JKI_lib_State_Machine.vi"("State(s) in (\"\")"=w278) -> ("States Out"=w277:string)  [unwired: 14 in]
      }
      frame "UI: Initialize" {
        w282 = "曲线编辑" ("前面板窗口:标题")
        w287 = u32 13816530
        # "树形清空"
        # "#CSM \"UI: Initialize\"\nInitialize the User Interface, here.\n(this is called automatically, by the Macro: Init)"
        n106 = control-ref of="循环树形"() -> (w279:refnum<vi>)
        n107 = control-ref of="窗格"() -> (w294:refnum<vi>)
        n108 = control-ref of="动作列表框"() -> (w289:refnum<vi>)
        n109 = local write "总时长[秒]"(0.0 ("总时长[秒]")) -> ()
        n110 = property class="Pane"(reference=w294, "Origin"=T4 {"Horizontal"=0, "Vertical"=0} ("原点")) -> ()  [unwired: 1 in, 2 out]
        n111 = property class="Tree (strict)"(reference=w279, "Allow Drop"=FALSE ("拖曳/放置:允许放置")) -> ()  [unwired: 1 in, 2 out]
        n112 = call "InitializeCurveList.vi"("循环树形"=w279, "ListBox输入"=w289) -> ("颜色符号列表"=w285:cluster{"项名":string, "颜色":u32, "符号":i32}[], "Tree引用输出"=w288:refnum<vi>)  [unwired: 6 in, 2 out]
        n113 = property class="Tree (strict)"(reference=w279, "SelColor"=w287) -> ()  [unwired: 1 in, 2 out]
        n114 = local write "曲线预览"(cluster{"X":dbl[], "Y":dbl[]} {"X"=[], "Y"=[]} ("曲线预览")) -> ()
        n115 = property on="动作列表框" class="LstBox (strict)"("SelColor"=w287) -> ()  [unwired: 2 in, 2 out]
        n116 = control-ref of="本VI"() -> (w283:refnum<vi>)
        n117 = invoke class="Tree (strict)" method="Edit Tree Items.Delete"(reference=w288) -> ()  [unwired: 4 in, 5 out]
        n118 = property class="VI"(reference=w283, "Front Panel.Title"=w282) -> (reference out=w280:refnum<vi>)  [unwired: 1 in, 1 out]
        n119 = Bundle By Name(cluster=w286, "User Data.颜色符号列表"=w285, "User Data.窗体标题"=w282) -> (w284:T9)
        n120 = control-ref of="Tab Control"() -> (w281:refnum<vi>)
        n121 = call "Match VI Window With TabControl.vi"("TabCtl Reference"=w281, "VI Reference"=w280) -> ()  [unwired: 10 in]
        n122 = call <vilib>:"Add State(s) to Queue__JKI_lib_State_Machine.vi"("State(s) in (\"\")"=w297) -> ("States Out"=w296:string)  [unwired: 14 in]
      }
      frame "UI: Cursor Set" {
        # "Argument"
        # "#CSM \"UI: Cursor Set\"\nSet and Unset Cursor Busy.\n(Usage: \"UI: Cursor Set >> Busy|Idle\")"
        n123 = disable-structure shown="Default" {
          disable-tunnel: [w305 _] -> w300
          disable-tunnel: w299 -> [w304 _]
          frame condition #0 (active) {
            n124 = case shown="\"Idle\", Default" w304 {
              tunnel: [w306 w307] -> w305
              frame "Idle", Default {
                n125 = call <vilib>:"Unset Busy.vi"() -> ("error out"=w306:errorcluster)  [unwired: 11 in]
              }
              frame "Busy" {
                n126 = call <vilib>:"Set Busy.vi"() -> ("error out"=w307:errorcluster)  [unwired: 10 in, 1 out]
              }
            }
          }
          frame condition #1 {
          }
        }
        n127 = call <vilib>:"Add State(s) to Queue__JKI_lib_State_Machine.vi"("State(s) in (\"\")"=w303) -> ("States Out"=w302:string)  [unwired: 14 in]
      }
      frame "UI: Front Panel State" {
        # "Argument"
        # "#CSM \"UI: Front Panel State\"\nSet Front Panel Open or Closed\n(Usage: \"UI: Front Panel State >> Open|Close\")"
        n128 = Unbundle By Name(w311) -> ("Core.Current VI Reference"=w310:refnum<vi>)
        n129 = case shown="\"Close\", \"Closed\"" w309 {
          tunnel: [w321 w334 w345 w357 w369] -> w312
          tunnel: w310 -> [w320 w332 w344 w356 w368]
          frame "Open", "Standard", Default {
            w315 = T1."Standard" ("State")
            n130 = property class="VI"(reference=w320) -> (reference out=w318:refnum<vi>, error out=w319:errorcluster, "FP.State"=w317:T1)  [unwired: 1 in]
            n131 = Not Equal?(x=w317, y=w315) -> (x != y?=w316:bool)
            n132 = case shown="True" w316 {
              tunnel: [w325 w327] -> w321
              tunnel: w319 -> [w324 w327]
              tunnel: w318 -> [w323 _]
              tunnel: w315 -> [w322 _]
              frame True {
                n133 = invoke class="VI" method="FP.Open"(reference=w323, error in=w324, "Activate"=TRUE, "State"=w322) -> (error out=w325:errorcluster)  [unwired: 1 in, 4 out]
              }
              frame False {
              }
            }
          }
          frame "Close", "Closed" {
            n134 = property class="VI"(reference=w332) -> (reference out=w331:refnum<vi>, error out=w333:errorcluster, "FP.State"=w329:T1)  [unwired: 1 in]
            n135 = Not Equal?(x=w329, y=T1."Closed" ("Front Panel Window:State")) -> (x != y?=w328:bool)
            n136 = case shown="True" w328 {
              tunnel: [w335 w338] -> w334
              tunnel: w333 -> [w335 w337]
              tunnel: w331 -> [_ w336]
              frame False {
              }
              frame True {
                n137 = invoke class="VI" method="FP.Close"(reference=w336, error in=w337) -> (error out=w338:errorcluster)  [unwired: 1 in, 2 out]
              }
            }
          }
          frame "Hidden", "Hide" {
            w339 = T1."Hidden" ("State")
            n138 = property class="VI"(reference=w344) -> (reference out=w342:refnum<vi>, error out=w343:errorcluster, "FP.State"=w341:T1)  [unwired: 1 in]
            n139 = Not Equal?(x=w341, y=w339) -> (x != y?=w340:bool)
            n140 = case shown="True" w340 {
              tunnel: [w349 w350] -> w345
              tunnel: w343 -> [w348 w350]
              tunnel: w342 -> [w347 _]
              tunnel: w339 -> [w346 _]
              frame True {
                n141 = invoke class="VI" method="FP.Open"(reference=w347, error in=w348, "State"=w346) -> (error out=w349:errorcluster)  [unwired: 2 in, 4 out]
              }
              frame False {
              }
            }
          }
          frame "Minimize", "Minimized" {
            w351 = T1."Minimized" ("State")
            n142 = property class="VI"(reference=w356) -> (reference out=w354:refnum<vi>, error out=w355:errorcluster, "FP.State"=w353:T1)  [unwired: 1 in]
            n143 = Not Equal?(x=w353, y=w351) -> (x != y?=w352:bool)
            n144 = case shown="False" w352 {
              tunnel: [w361 w362] -> w357
              tunnel: w355 -> [w360 w362]
              tunnel: w354 -> [w359 _]
              tunnel: w351 -> [w358 _]
              frame True {
                n145 = invoke class="VI" method="FP.Open"(reference=w359, error in=w360, "State"=w358) -> (error out=w361:errorcluster)  [unwired: 2 in, 4 out]
              }
              frame False {
              }
            }
          }
          frame "Maximize", "Maximized" {
            w363 = T1."Maximized" ("State")
            n146 = property class="VI"(reference=w368) -> (reference out=w366:refnum<vi>, error out=w367:errorcluster, "FP.State"=w365:T1)  [unwired: 1 in]
            n147 = Not Equal?(x=w365, y=w363) -> (x != y?=w364:bool)
            n148 = case shown="True" w364 {
              tunnel: [w373 w374] -> w369
              tunnel: w367 -> [w372 w374]
              tunnel: w366 -> [w371 _]
              tunnel: w363 -> [w370 _]
              frame True {
                n149 = invoke class="VI" method="FP.Open"(reference=w371, error in=w372, "State"=w370) -> (error out=w373:errorcluster)  [unwired: 2 in, 4 out]
              }
              frame False {
              }
            }
          }
        }
        n150 = call <vilib>:"Add State(s) to Queue__JKI_lib_State_Machine.vi"("State(s) in (\"\")"=w314) -> ("States Out"=w313:string)  [unwired: 14 in]
      }
      frame "---------- Macro ----------" {
        # "#CSM \"Category Seperator\"\nDo not put any code in this frame."
        n151 = call <vilib>:"Add State(s) to Queue__JKI_lib_State_Machine.vi"("State(s) in (\"\")"=w378) -> ("States Out"=w377:string)  [unwired: 14 in]
      }
      frame "Macro: Initialize" {
        w380 = "Data: Initialize\nInitialize Core Data\nEvents: Register\nUI: Initialize\nUI: Front Panel State >> Open"  # Data: Initialize Initialize Core Data Events: Register UI: Initialize UI: Front Panel State >> Open
        # "#CSM \"Macro: Initialize\"\nInitialization Macro (This is called once, when the VI starts)"
        n152 = call <vilib>:"Add State(s) to Queue__JKI_lib_State_Machine.vi"("State(s) in Front (\"\")"=w380, "State(s) in (\"\")"=w383) -> ("States Out"=w382:string)  [unwired: 13 in]
      }
      frame "Macro: Exit" {
        # "#CSM \"Macro: Exit\"\nExit Macro (This is called once, when the VI exits)"
        n153 = Unbundle By Name(w392) -> ("Core.Close Panel on Exit?"=w391:bool)
        n154 = Select(t="UI: Front Panel State >> Close", s=w391, f="") -> (s? t:f=w388:string)
        n155 = call <vilib>:"Add State(s) to Queue__JKI_lib_State_Machine.vi"("State(s) in Front (\"\")"="//Exit Sub-Modules ", "State(s) in (\"\")"=w388, "State(s) at Back (\"\")"="Data: Cleanup\nEvents: Unregister\nExit") -> ("States Out"=w386:string)  [unwired: 12 in]
        n156 = call <vilib>:"Add State(s) to Queue__JKI_lib_State_Machine.vi"("State(s) in Front (\"\")"=w386, "State(s) in (\"\")"=w394) -> ("States Out"=w393:string)  [unwired: 13 in]
      }
      frame "---------- API ----------" {
        # "#CSM \"Category Seperator\"\nDo not put any code in this frame."
      }
      frame "API: Open File" {
        # "#CSM \"Category Seperator\"\nDo not put any code in this frame."
        n157 = String To Path(string=w403) -> (path=w401:path)
        n158 = Bundle By Name(cluster=w405, "User Data.文件路径"=w401) -> (w402:T9)
        n159 = call <vilib>:"Add State(s) to Queue__jki_lib_state_machine.vi"("State(s) in (\"\")"=w399, "State(s) at Back (\"\")"="Action: Read File" ("State(s) at Back (\"\")")) -> ("States Out"=w400:string)  [unwired: 13 in]
      }
      frame "---------- Action ----------" {
        # "#CSM \"Category Seperator\"\nDo not put any code in this frame."
        n160 = call <vilib>:"Add State(s) to Queue__JKI_lib_State_Machine.vi"("State(s) in (\"\")"=w409) -> ("States Out"=w408:string)  [unwired: 14 in]
      }
      frame "Action: Write File" {
        # "#CSM \"Internal State\"\nThis category is used for holding internal states"
        n161 = Unbundle By Name(w410) -> ("User Data.存盘提醒"=w412:bool, "User Data.文件路径"=w414:path, "User Data.窗体标题"=w413:string, "User Data.循环数组"=w415:string[])
        n162 = for {
          tunnel: w415 -> [w445] mode=indexing
          shift-right: [w442] -> w421
          shift-left: "" -> [w443]
          i -> [w450]
          # "将字符串数组转换为换行符分隔的字符串"
          n163 = Equal To 0?(x=w450) -> (x = 0?=w449:bool)
          n164 = Select(t="", s=w449, f="\n") -> (s? t:f=w446:string)
          n165 = Concatenate Strings(w446, w445) -> (w444:string)
          n166 = Concatenate Strings(w443, w444) -> (w442:string)
        }
        n167 = Open/Create/Replace File(file path (use dialog)=w414, operation (0:open)=T5."replace or create" ("操作(0:open)"), access (0:read/write)=enum16{"read/write", "read-only", "write-only"}."write-only" ("权限(0:read/write)")) -> (refnum out=w418:refnum<file>, error out=w419:errorcluster)  [unwired: 3 in, 1 out]
        n168 = Write to Text File(file (use dialog)=w418, text=w421, error in=w419) -> (refnum out=w422:refnum<file>, error out=w423:errorcluster)  [unwired: 1 in, 1 out]
        n169 = Close File(refnum=w422, error in=w423) -> (path=w425:path, error out=w424:errorcluster)
        n170 = case shown="No Error" w424 {
          tunnel: w425 -> [w434 _]
          tunnel: w413 -> [w433 _]
          tunnel: w412 -> [w432 _]
          tunnel: w410 -> [w431 w440]
          tunnel: [w429 w440] -> w411
          frame No Error {
            n171 = call <vilib>:"Get File Extension.vi"("file"=w434) -> ("filename without extension"=w436:string)  [unwired: 6 in, 4 out]
            n172 = Bundle By Name(cluster=w431, "User Data.文件已保存"=TRUE ("文件已保存")) -> (w429:T9)
            n173 = case shown="True" w432 {
              frame False {
              }
              frame True {
                n174 = One Button Dialog(message="文件保存成功！" ("消息")) -> ()  [unwired: 1 in, 1 out]
              }
            }
            n175 = control-ref of="本VI"() -> (w435:refnum<vi>)
            n176 = Concatenate Strings(w436, " - " ("字符串"), w433) -> (w438:string)
            n177 = property class="VI"(reference=w435, "Front Panel.Title"=w438) -> ()  [unwired: 1 in, 2 out]
          }
          frame Error {
            n178 = One Button Dialog(message="文件保存失败！" ("消息")) -> ()  [unwired: 1 in, 1 out]
          }
        }
        n179 = call <vilib>:"Add State(s) to Queue__JKI_lib_State_Machine.vi"("State(s) in (\"\")"=w428) -> ("States Out"=w427:string)  [unwired: 14 in]
      }
      frame "Action: Read File" {
        # "#CSM \"Internal State\"\nThis category is used for holding internal states"
        n180 = Unbundle By Name(w454) -> ("User Data.文件路径"=w458:path, "User Data.颜色符号列表"=w457:cluster{"项名":string, "颜色":u32, "符号":i32}[], "User Data.窗体标题"=w456:string)
        n181 = call-poly <vilib>:"Read Delimited Spreadsheet.vi"("file path (dialog if empty)"=w458) -> ("all rows"=w453:string[][])  [unwired: 9 in, 5 out]
        n182 = Index Array(array=w453, index (col)=0 ("禁用的索引 (列)")) -> (element=w461:string[])  [unwired: 1 in]
        n183 = control-ref of="循环树形"() -> (w460:refnum<vi>)
        n184 = call "Array2Tree.vi"("颜色符号列表"=w457, "循环数组"=w461, "循环树形引用输入"=w460) -> ("错误输出"=w462:errorcluster, "循环树形引用输出"=w463:refnum<vi>)  [unwired: 7 in]
        n185 = case shown="No Error" w462 {
          tunnel: w458 -> [w466 _]
          tunnel: w463 -> [w474 _]
          tunnel: w456 -> [w473 _]
          tunnel: w454 -> [w472 w481]
          tunnel: [w469 w481] -> w455
          tunnel: w452 -> [w468 w480]
          tunnel: [w467 w480] -> w451
          frame No Error {
            n186 = call <vilib>:"Get File Extension.vi"("file"=w466) -> ("filename without extension"=w476:string)  [unwired: 6 in, 4 out]
            n187 = call "Tree2Array.vi"("TreeControl输入"=w474) -> ("循环数组"=w470:string[])  [unwired: 9 in, 1 out]
            n188 = Bundle By Name(cluster=w472, "User Data.文件已保存"=TRUE ("文件已保存"), "User Data.循环数组"=w470) -> (w469:T9)
            n189 = control-ref of="本VI"() -> (w475:refnum<vi>)
            n190 = call <vilib>:"Add State(s) to Queue__JKI_lib_State_Machine.vi"("State(s) in (\"\")"=w468, "State(s) at Back (\"\")"="Action: Draw Plot" ("State(s) at Back (\"\")")) -> ("States Out"=w467:string)  [unwired: 13 in]
            n191 = Concatenate Strings(w476, " - " ("字符串"), w473) -> (w478:string)
            n192 = property class="VI"(reference=w475, "Front Panel.Title"=w478) -> ()  [unwired: 1 in, 2 out]
          }
          frame Error {
            n193 = One Button Dialog(message="文件错误！") -> ()  [unwired: 1 in, 1 out]
          }
        }
      }
      frame "Action: Draw Plot" {
        n194 = Unbundle By Name(w483) -> ("User Data.循环数组"=w482:string[])
        n195 = call "DrawCurve.vi"("曲线定义数组"=w482) -> ("曲线输出"=w488:cluster{"X":dbl[], "Y":dbl[]})  [unwired: 10 in]
        "曲线预览" <- w488
        n196 = Unbundle(w488) -> ("X"=w487:dbl[])  [unwired: 1 out]
        n197 = Delete From Array(array=w487, length=1 ("长度")) -> (deleted portion=w486:dbl[])  [unwired: 1 in, 1 out]
        n198 = Index Array(array=w486) -> (element=→"总时长[秒]":dbl)  [unwired: 1 in]
      }
      frame "Action: Handle Unsaved Porcess" {
        n199 = Two Button Dialog(message="是否保存现有文件？" ("消息"), 1:"不保存" ("F按钮名称（“取消”）"), 2:"保存" ("T按钮名称（“确定”）")) -> (T button?=w499:bool)
        n200 = case shown="True" w499 {
          tunnel: [w503 w509] -> w495
          tunnel: w494 -> [w504 w510]
          tunnel: [w505 w508] -> w493
          tunnel: w492 -> [w505 w507]
          frame False {
            n201 = Bundle By Name(cluster=w504, "User Data.文件已保存"=TRUE ("新建按钮")) -> (w503:T9)
          }
          frame True {
            # "文件要保存"
            n202 = Unbundle By Name(w510) -> ("User Data.文件路径"=w511:path, "User Data.文件参数"=w506:T11)
            n203 = control-ref of="本VI"() -> (w514:refnum<vi>)
            n204 = call "SaveFileDialogue.vi"("文件参数"=w506, "文件路径"=w511, "VI输入"=w514) -> ("错误输出"=w513:errorcluster, "输出路径"=w512:path)  [unwired: 6 in, 1 out]
            n205 = case shown="No Error" w513 {
              tunnel: w512 -> [w521 _]
              tunnel: [w518 w524] -> w509
              tunnel: w510 -> [w522 w524]
              tunnel: [w516 w523] -> w508
              tunnel: w507 -> [w517 w523]
              frame No Error {
                n206 = control-ref of="循环树形"() -> (w520:refnum<vi>)
                n207 = call "Tree2Array.vi"("TreeControl输入"=w520) -> ("循环数组"=w519:string[])  [unwired: 9 in, 1 out]
                n208 = Bundle By Name(cluster=w522, "User Data.文件路径"=w521, "User Data.循环数组"=w519) -> (w518:T9)
                n209 = call <vilib>:"Add State(s) to Queue__JKI_lib_State_Machine.vi"("State(s) in Front (\"\")"="Action: Write File" ("State(s) in Front (\"\")"), "State(s) in (\"\")"=w517) -> ("States Out"=w516:string)  [unwired: 13 in]
              }
              frame Error {
              }
            }
          }
        }
      }
      frame "Action: Open File" {
        n210 = Unbundle By Name(w528) -> ("User Data.文件参数"=w529:T11)
        n211 = Unbundle By Name(w529) -> ("默认路径"=w532:path, "类型(后缀名)"=w531:string, "类型标签"=w530:string)
        n212 = call "文件对话框"("start path"=w532, "pattern (all files)"=w531, "pattern label"=w530) -> ("selected path"=w533:path, "exists"=w535:bool, "error out"=w534:errorcluster)  [unwired: 9 in, 1 out]
        n213 = case shown="No Error" w534 {
          tunnel: w533 -> [w542 _]
          tunnel: w535 -> [w543 _]
          tunnel: w528 -> [w540 w553]
          tunnel: w527 -> [w538 w552]
          tunnel: [w541 w553] -> w526
          tunnel: [w539 w552] -> w525
          frame No Error {
            n214 = case shown="True" w543 {
              tunnel: w542 -> [_ w549]
              tunnel: [w545 w550] -> w541
              tunnel: w540 -> [w545 w551]
              tunnel: [w544 w547] -> w539
              tunnel: w538 -> [w544 w548]
              frame False {
              }
              frame True {
                n215 = Bundle By Name(cluster=w551, "User Data.文件路径"=w549) -> (w550:T9)
                n216 = call <vilib>:"Add State(s) to Queue__JKI_lib_State_Machine.vi"("State(s) in (\"\")"=w548, "State(s) at Back (\"\")"="Action: Read File" ("State(s) at Back (\"\")")) -> ("States Out"=w547:string)  [unwired: 13 in]
              }
            }
          }
          frame Error {
          }
        }
      }
      frame "Action: Save File" {
        n217 = Unbundle By Name(w558) -> ("User Data.文件参数"=w557:T11)
        n218 = call "Convert API String Arguments to Data.vim"("Reference Type"=path "", "API String"=w556) -> ("Data"=w555:path)  [unwired: 6 in, 1 out]
        n219 = control-ref of="本VI"() -> (w562:refnum<vi>)
        n220 = call "SaveFileDialogue.vi"("文件参数"=w557, "文件路径"=w555, "VI输入"=w562) -> ("错误输出"=w564:errorcluster, "输出路径"=w563:path)  [unwired: 6 in, 1 out]
        n221 = case shown="No Error" w564 {
          tunnel: w563 -> [w571 _]
          tunnel: w558 -> [w573 w576]
          tunnel: [w572 w576] -> w561
          tunnel: [w569 w575] -> w560
          tunnel: w559 -> [w568 w575]
          frame No Error {
            n222 = control-ref of="循环树形"() -> (w574:refnum<vi>)
            n223 = call "Tree2Array.vi"("TreeControl输入"=w574) -> ("循环数组"=w570:string[])  [unwired: 9 in, 1 out]
            n224 = Bundle By Name(cluster=w573, "User Data.文件路径"=w571, "User Data.循环数组"=w570) -> (w572:T9)
            n225 = call <vilib>:"Add State(s) to Queue__JKI_lib_State_Machine.vi"("State(s) in (\"\")"=w568, "State(s) at Back (\"\")"="Action: Write File" ("State(s) at Back (\"\")")) -> ("States Out"=w569:string)  [unwired: 13 in]
          }
          frame Error {
          }
        }
      }
      frame "Action: New File" {
        w584 = "曲线" ("左单元格字符串")
        n226 = control-ref of="循环树形"() -> (w595:refnum<vi>)
        n227 = Unbundle By Name(w579) -> ("User Data.文件参数"=w578:T11, "User Data.窗体标题"=w577:string)
        n228 = invoke class="Tree (strict)" method="Edit Tree Items.Delete"(reference=w595) -> (reference out=w591:refnum<vi>)  [unwired: 4 in, 4 out]
        n229 = control-ref of="本VI"() -> (w594:refnum<vi>)
        n230 = invoke class="Tree (strict)" method="Edit Tree Items.Add Item"(reference=w591, "Child Position"=-1 ("子项位置"), "Left Cell"=w584, "Child Tag"=w584) -> (reference out=w590:refnum<vi>, "Edit Tree Items:Add Item"=w589:string)  [unwired: 5 in, 7 out]
        n231 = Unbundle By Name(w578) -> ("默认名称"=w592:string)
        n232 = Concatenate Strings(w592, " - " ("字符串"), w577) -> (w593:string)
        n233 = property class="VI"(reference=w594, "Front Panel.Title"=w593) -> ()  [unwired: 1 in, 2 out]
        n234 = call "Tree2Array.vi"("TreeControl输入"=w590) -> ("循环数组"=w580:string[])  [unwired: 9 in, 1 out]
        n235 = property class="Tree (strict)"(reference=w590, "Active Item Tag"=w589, "Glyph"=1 ("活动项:符号索引")) -> ()  [unwired: 1 in, 2 out]
        n236 = Bundle By Name(cluster=w579, "User Data.文件路径"=path "", "User Data.循环数组"=w580) -> (w582:T9)
        n237 = local write "总时长[秒]"(0.0 ("总时长[秒]")) -> ()
        n238 = local write "曲线预览"(cluster{"X":dbl[], "Y":dbl[]} {"X"=[], "Y"=[]} ("曲线预览")) -> ()
        n239 = call <vilib>:"Add State(s) to Queue__JKI_lib_State_Machine.vi"("State(s) in (\"\")"=w598) -> ("States Out"=w597:string)  [unwired: 14 in]
      }
      frame "Action: Edit Item" {
        # "通过标识获取行索引和首列文本"
        n240 = control-ref of="循环树形"() -> (w604:refnum<vi>)
        n241 = property class="Tree (strict)"(reference=w604, "ActiveColNum"=0 ("活动单元格:活动列数")) -> (reference out=w607:refnum<vi>, error out=w606:errorcluster, "Active Item Row Number"=w608:i32, "Indent Level"=w609:i32, "Cell String"=w605:string)  [unwired: 1 in]
        n242 = case shown="No Error" w606 {
          selector: w606 -> [_ w641]
          tunnel: w605 -> [w620 _]
          tunnel: w607 -> [w619 _]
          tunnel: w608 -> [w618 _]
          tunnel: w609 -> [w617 _]
          tunnel: [w615 w640] -> w602
          tunnel: w601 -> [w614 w640]
          tunnel: [w613 w639] -> w600
          tunnel: w599 -> [w612 w639]
          frame No Error {
            n243 = Not Equal To 0?(x=w617) -> (x != 0?=w616:bool)
            n244 = case shown="True" w616 {
              tunnel: w620 -> [_ w634]
              tunnel: w619 -> [_ w633]
              tunnel: w618 -> [_ w630]
              tunnel: [w622 w628] -> w615
              tunnel: w614 -> [w622 w629]
              tunnel: [w621 w625] -> w613
              tunnel: w612 -> [w621 w624]
              frame False {
              }
              frame True {
                # "编辑窗打开，文件变为未保存"
                # "打开编辑窗口"
                # "动作选择"
                # "当为子项时打开编辑窗口"
                n245 = case shown="\"抛物线\"" w634 {
                  tunnel: [w635 w636 w637 w638] -> w631
                  frame "假", Default {
                    n246 = vi-ref "EditLine.vi"() -> (w635:refnum<vi>)
                  }
                  frame "直线" {
                    n247 = vi-ref "EditLine.vi"() -> (w636:refnum<vi>)
                  }
                  frame "正弦" {
                    n248 = vi-ref "EditSine.vi"() -> (w637:refnum<vi>)
                  }
                  frame "抛物线" {
                    n249 = vi-ref "EditParabola.vi"() -> (w638:refnum<vi>)
                  }
                }
                n250 = call "CallEditVI.vi"("VI引用句柄"=w631, "索引"=w630, "TreeControl输入"=w633) -> ("TreeControl输出"=w632:refnum<vi>)  [unwired: 7 in, 1 out]
                n251 = call "Tree2Array.vi"("TreeControl输入"=w632) -> ("循环数组"=w627:string[])  [unwired: 9 in, 1 out]
                n252 = Bundle By Name(cluster=w629, "User Data.循环数组"=w627, "User Data.文件已保存"=FALSE ("文件已保存")) -> (w628:T9)
                n253 = call <vilib>:"Add State(s) to Queue__JKI_lib_State_Machine.vi"("State(s) in (\"\")"=w624, "State(s) at Back (\"\")"="Action: Draw Plot" ("State(s) at Back (\"\")")) -> ("States Out"=w625:string)  [unwired: 13 in]
              }
            }
          }
          frame Error {
            n254 = call <vilib>:"Clear Errors.vi"("error in (no error)"=w641) -> ()  [unwired: 5 in, 2 out]
          }
        }
      }
    }
  }
